vi "Wait UI.vi"(8 "error in (no error)":errorcluster, 9 "Timeout [mSec] (-1)":i32=-1, 11 "Bar in":refnum<class "Bar.lvclass">) -> (0 "error out":errorcluster, 1 "Timed Out ?":bool, 2 "No Wait ?":bool, 3 "Bar out":refnum<class "Bar.lvclass">)   [LabVIEW 2015, in "Simple Progress Bar.lvlib" / "Bar.lvclass"]
doc: "Wait the progress bar user interface to be closed by the user or automatically."
uses:
  Bar.lvclass
  Bar.lvclass/Bar.ctl
panel:
  out "Waiting for User":bool
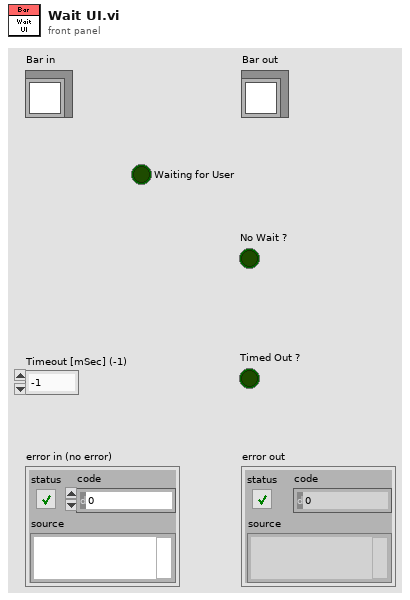
[diagram p1: front panel]
types:
  T1 = enum32{"Invalid", "Standard", "Closed", "Hidden", "Minimized", "Maximized"}
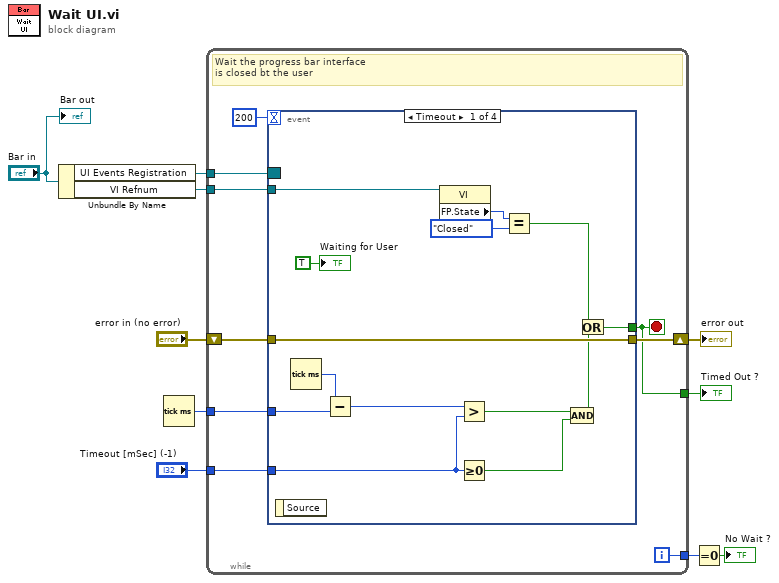
[diagram p0: block diagram]
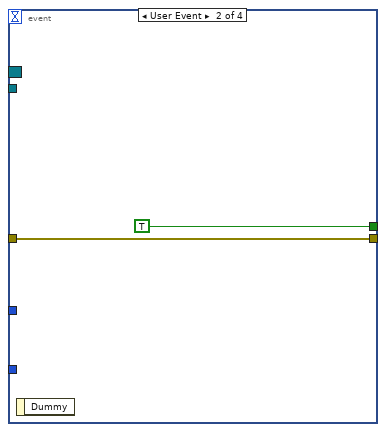
[diagram p2: hidden frame]
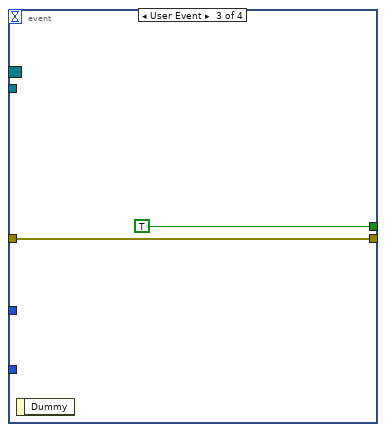
[diagram p3: hidden frame]
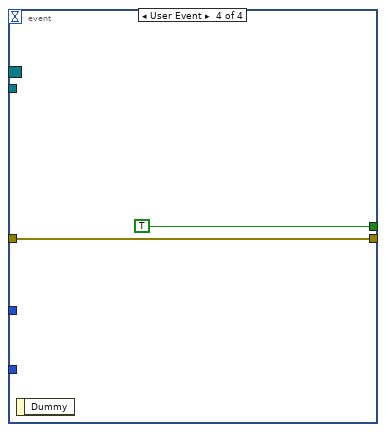
[diagram p4: hidden frame]
diagram:
  n1 = Unbundle By Name("Bar in") -> ("UI Events Registration"=w3:refnum<event-registration>, "VI Refnum"=w1:refnum<vi>)
  n2 = Tick Count (ms)() -> (millisecond timer value=w8:u32)
  n3 = while {
    shift-right: [w18] -> w9
    shift-left: "error in (no error)" -> [w19]
    tunnel: w3 -> [w16]
    tunnel: w8 -> [w15]
    tunnel: "Timeout [mSec] (-1)" -> [w14]
    tunnel: [w13] -> w6
    tunnel: [w12] -> w5
    tunnel: w1 -> [w11]
    i -> [w12]
    stop <- w13 stop-if-true
    # "Wait the progress bar interface\nis closed bt the user"
    n4 = event shown="[0] Timeout" {
      selector: w16 -> [_ _ _ _]
      dyn-events: _ -> [_ _ _ _]
      timeout: 200 -> [_ _ _ _]
      tunnel: [w33 w35 w36 w38] -> w18
      tunnel: w19 -> [w33 w35 w36 w38]
      tunnel: [w21 TRUE TRUE TRUE] -> w13
      tunnel: w15 -> [w30 _ _ _]
      tunnel: w14 -> [w26 _ _ _]
      tunnel: w11 -> [w24 _ _ _]
      event Timeout {
        n5 = event-data() -> ()  [unwired: 1 in, 1 out]
        n6 = Tick Count (ms)() -> (millisecond timer value=w31:u32)
        n7 = Subtract(x=w31, y=w30) -> (x-y=w29:u32)
        n8 = property class="VI"(reference=w24) -> ("FP.State"=w23:T1)  [unwired: 1 in, 2 out]
        n9 = Greater?(x=w29, y=w26) -> (0:w28:bool)
        n10 = Greater Or Equal To 0?(x=w26) -> (x >= 0?=w25:bool)
        n11 = Equal?(x=w23, y=T1."Closed") -> (x = y?=w20:bool)
        n12 = Compound Arithmetic op=AND(w28, w25) -> (w27:bool)
        n13 = Or(x=w20, y=w27) -> (x .or. y?=w21:bool)
        "Waiting for User" <- TRUE ("Waiting for User")
      }
      event User Event {
        n14 = event-data() -> ()  [unwired: 1 in, 1 out]
      }
      event User Event {
        n15 = event-data() -> ()  [unwired: 1 in, 1 out]
      }
      event User Event {
        n16 = event-data() -> ()  [unwired: 1 in, 1 out]
      }
    }
  }
  "error out" <- w9
  "Timed Out ?" <- w6
  n17 = Equal To 0?(x=w5) -> (x = 0?=→"No Wait ?":bool)
  "Bar out" <- "Bar in"
